vi "[ex ce] CE Server Example.vi"() -> ()   [LabVIEW 2021]
doc: "<B>CE Server Example</B>\n\nThis is simplest example of a server VI to execute requests to CalcExpress VIs from remote or local clients.\n\n::: CalcExpress Toolkit :::\nCopyright (c) 2000-2026 Konstantin Shifershteyn. All rights reserved."
panel:
  in  "False":bool
  in  "Allow TCP access":bool=TRUE
  in  "stop":bool
  in  "TCP access list":string[](array[string])=["localdomain"]
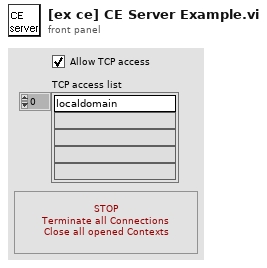
[diagram p1: front panel]
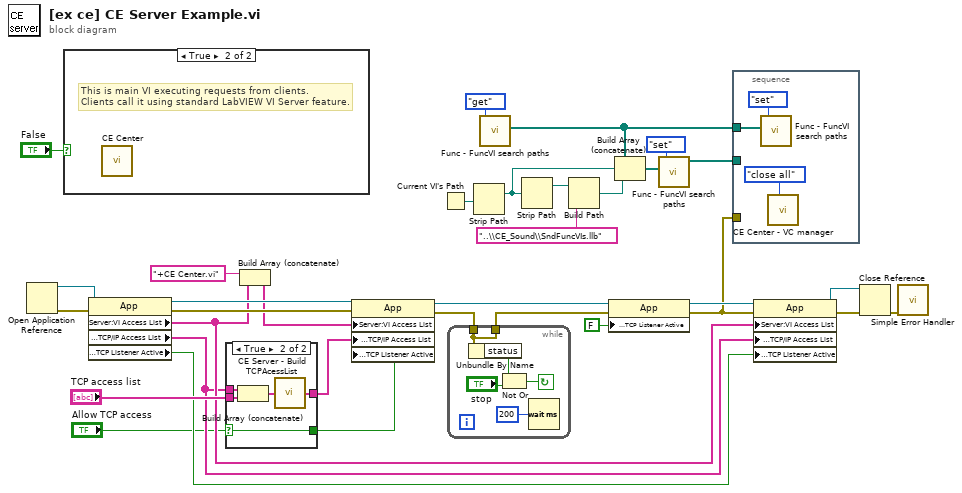
[diagram p0: block diagram]
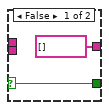
[diagram p2: hidden frame]
diagram:
  n1 = Open Application Reference() -> (0:w32:errorcluster, 3:w33:refnum<vi>)  [unwired: 4 in]
  n2 = case shown="True" "False" {
    frame False {
    }
    frame True {
      # "This is main VI executing requests from clients.\nClients call it using standard LabVIEW VI Server feature."
      n3 = call "CE Center.vi"() -> ()  [unwired: 9 in, 3 out]
    }
  }
  n4 = property class="App"(reference=w33, error in=w32) -> (reference out=w31:refnum<vi>, error out=w30:errorcluster, "Server:VI Access List"=w7:string[], "Server:TCP/IP Access List"=w6:string[], "Server:TCP Listener Active"=w22:bool)
  n5 = case shown="True" "Allow TCP access" {
    selector: "Allow TCP access" -> [w35 w36]
    tunnel: "TCP access list" -> [_ w39]
    tunnel: w6 -> [_ w38]
    tunnel: [string[] [] ("TCPAccessList out") w37] -> w5
    tunnel: [w35 w36] -> w3
    frame False {
    }
    frame True {
      n6 = Build Array (concatenate)(w38, w39) -> (w40:string[])
      n7 = call "CE Server - Build TCPAcessList.vi"("TCPAccessList in"=w40) -> ("TCPAccessList out"=w37:string[])
    }
  }
  n8 = Build Array (concatenate)("+CE Center.vi", w7) -> (w29:string[])
  n9 = property class="App"(reference=w31, error in=w30, "Server:VI Access List"=w29, "Server:TCP/IP Access List"=w5, "Server:TCP Listener Active"=w3) -> (reference out=w26:refnum<vi>, error out=w2:errorcluster)
  n10 = Current VI's Path() -> (path=w17:path)
  n11 = while {
    tunnel: [w41] -> w1
    tunnel: w2 -> [w41]
    stop <- w45 continue-if-true
    n12 = Unbundle By Name(w41) -> ("status"=w43:bool)
    n13 = Not Or(1:"stop", 2:w43) -> (0:w45:bool)
    n14 = Wait (ms)(milliseconds to wait=u32 200) -> ()  [unwired: 1 out]
  }
  n15 = Strip Path(path=w17) -> (stripped path=w12:path)  [unwired: 1 out]
  n16 = call "Func - FuncVI search paths.vi"("cmd"=enum16{"get", "set"}."get") -> ("user paths out"=w15:path[])  [unwired: 5 in, 3 out]
  n17 = Strip Path(path=w12) -> (stripped path=w16:path)  [unwired: 1 out]
  n18 = Build Path(base path=w16, name or relative path="..\\CE_Sound\\SndFuncVIs.llb") -> (appended path=w11:path)
  n19 = property class="App"(reference=w26, error in=w1, "Server:TCP Listener Active"=FALSE ("Srvr.TCPActive")) -> (reference out=w25:refnum<vi>, error out=w9:errorcluster)
  n20 = Build Array (concatenate)(w15, w12, w11) -> (w18:path[])
  n21 = call "Func - FuncVI search paths.vi"("cmd"=enum16{"get", "set"}."set", "user paths"=w18) -> ("search paths"=w13:path[])  [unwired: 4 in, 3 out]
  n22 = stacked-sequence {
    tunnel: w15 -> [w46]
    tunnel: w9 -> [_]
    tunnel: w13 -> [_]
    frame #0 {
      n23 = call "Func - FuncVI search paths.vi"("cmd"=enum16{"get", "set"}."set", "user paths"=w46) -> ()  [unwired: 4 in, 4 out]
      n24 = call "CE Center - VC manager.vi"("cmd"=enum16{"open", "close", "close all"}."close all") -> ()  [unwired: 6 in, 3 out]
    }
  }
  n25 = property class="App"(reference=w25, error in=w9, "Server:VI Access List"=w7, "Server:TCP/IP Access List"=w6, "Server:TCP Listener Active"=w22) -> (reference out=w24:refnum<vi>, error out=w8:errorcluster)
  n26 = Close Reference(reference=w24, error in (no error)=w8) -> (error out=w10:errorcluster)
  n27 = call <vilib>:"Simple Error Handler.vi"("error in (no error)"=w10) -> ()  [unwired: 4 in, 5 out]
